vi "ZM-TST-pipeline.vi"() -> (0 "error out":errorcluster, 3 "Pass":bool)   [LabVIEW 2020, in "ZM-TST-tests.lvlib"]
doc: "T6, the data path without actors: simulated hardware into a file logger for 10 packages, after which TestPackage.jsonl holds 10 valid lines (pipeline_ok); with the placeholder hardware the first do fails and nothing is written (error_stops_ok). Pass = AND of both. Side effect: two temp folders under output."
uses:
  ZM-TST-tests.lvlib
  hardware/ZM-HW-SIM-simulated_hardware/ZM-HW-SIM-simulated_hardware/ZM-HW-SIM-simulated_hardware.lvclass
  hardware/ZM-HW-hardware/ZM-HW-hardware/ZM-HW-hardware.lvclass
  protocol/ZM-CP-FL-file_logger/ZM-CP-FL-file_logger/ZM-CP-FL-file_logger.lvclass
panel:
  out "error_stops_ok":bool
  out "pipeline_ok":bool
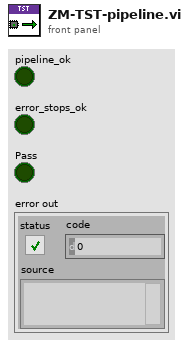
[diagram p1: front panel]
types:
  T1 = cluster{"timestamp":string, "type":string, "destination":string, "data":cluster{"temperature_c":dbl, "sample_index":i32, "duty_percent":u8, "sensor_ok":bool, "status":string}}
  T2 = cluster{"temperature_c":dbl, "sample_index":i32, "duty_percent":u8, "sensor_ok":bool, "status":string}
  T3 = cluster{"temperature_c":bool, "sample_index":bool, "duty_percent":bool, "sensor_ok":bool, "status":bool}
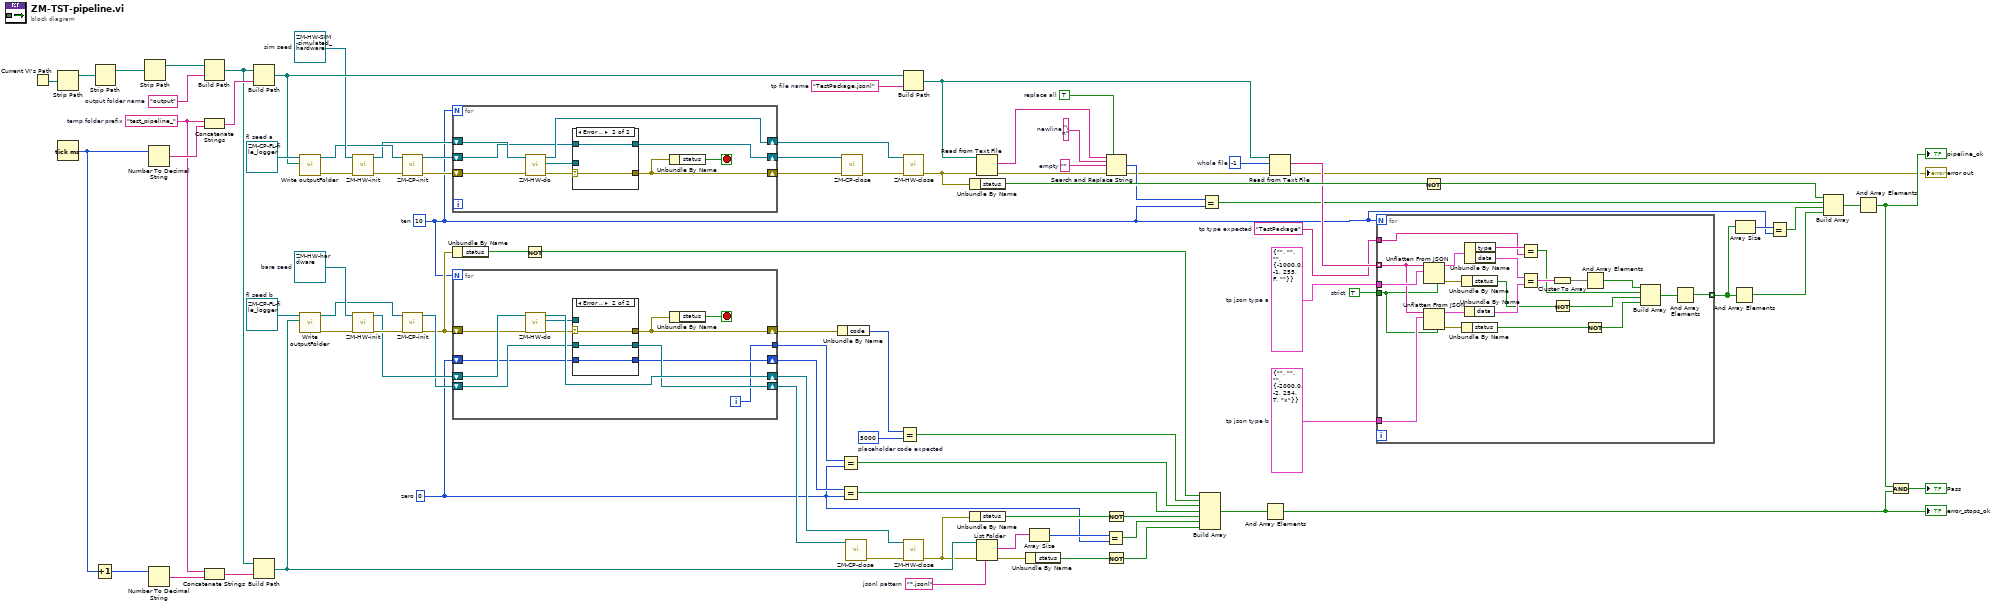
[diagram p0: block diagram]
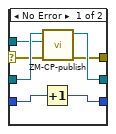
[diagram p2: hidden frame]
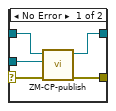
[diagram p3: hidden frame]
diagram:
  w15 = 0  # zero
  w18 = "*.jsonl"  # jsonl pattern
  w27 = 5000  # placeholder code expected
  w48 = TRUE  # strict
  w49 = T1 {"timestamp"="", "type"="", "destination"="", "data"={"temperature_c"=-2000.0, "sample_index"=-2, "duty_percent"=254, "sensor_ok"=TRUE, "status"="x"}}  # tp json type b
  w50 = T1 {"timestamp"="", "type"="", "destination"="", "data"={"temperature_c"=-1000.0, "sample_index"=-1, "duty_percent"=255, "sensor_ok"=FALSE, "status"=""}}  # tp json type a
  w30 = 10  # ten
  w53 = -1  # whole file
  w56 = TRUE  # replace all
  w58 = ""  # empty
  w59 = "\n"  # newline
  w47 = "TestPackage"  # tp type expected
  w76 = "TestPackage.jsonl"  # tp file name
  w86 = "test_pipeline_"  # temp folder prefix
  w80 = "output"  # output folder name
  w39 = refnum<class "ZM-CP-FL-file_logger.lvclass"> refnum  # fl seed b
  w75 = refnum<class "ZM-CP-FL-file_logger.lvclass"> refnum  # fl seed a
  w38 = refnum<class "ZM-HW-hardware.lvclass"> refnum  # bare seed
  w73 = refnum<class "ZM-HW-SIM-simulated_hardware.lvclass"> refnum  # sim seed
  n1 = Current VI's Path() -> (path=w84:path)
  n2 = Strip Path(path=w84) -> (stripped path=w83:path)  [unwired: 1 out]
  n3 = Tick Count (ms)() -> (millisecond timer value=w88:u32)
  n4 = Increment(x=w88) -> (x+1=w87:u32)
  n5 = Strip Path(path=w83) -> (stripped path=w82:path)  [unwired: 1 out]
  n6 = Strip Path(path=w82) -> (stripped path=w81:path)  [unwired: 1 out]
  n7 = Number To Decimal String(number=w88) -> (decimal integer string=w89:string)  [unwired: 1 in]
  n8 = Number To Decimal String(number=w87) -> (decimal integer string=w85:string)  [unwired: 1 in]
  n9 = Build Path(base path=w81, name or relative path=w80) -> (appended path=w78:path)
  n10 = Concatenate Strings(w86, w89) -> (w79:string)
  n11 = Concatenate Strings(w86, w85) -> (w77:string)
  n12 = Build Path(base path=w78, name or relative path=w79) -> (appended path=w74:path)
  n13 = Build Path(base path=w78, name or relative path=w77) -> (appended path=w20:path)
  n14 = call "Write outputFolder.vi"("outputFolder"=w74, "ZM-CP-FL-file_logger in"=w75) -> ("error out"=w72:errorcluster, "ZM-CP-FL-file_logger out"=w71:refnum<class "ZM-CP-FL-file_logger.lvclass">)  [unwired: 8 in]
  n15 = call "Write outputFolder.vi"("outputFolder"=w20, "ZM-CP-FL-file_logger in"=w39) -> ("error out"=w37:errorcluster, "ZM-CP-FL-file_logger out"=w36:refnum<class "ZM-CP-FL-file_logger.lvclass">)  [unwired: 8 in]
  n16 = call-dynamic "ZM-HW-init.vi"("error in (no error)"=w72, "ZM-HW-hardware in"=w73) -> ("error out"=w70:errorcluster, "ZM-HW-hardware out"=w69:refnum<class "ZM-HW-SIM-simulated_hardware.lvclass">)  [unwired: 8 in]
  n17 = call-dynamic "ZM-HW-init.vi"("error in (no error)"=w37, "ZM-HW-hardware in"=w38) -> ("error out"=w35:errorcluster, "ZM-HW-hardware out"=w33:refnum<class "ZM-HW-hardware.lvclass">)  [unwired: 8 in]
  n18 = call-dynamic "ZM-CP-init.vi"("error in (no error)"=w70, "ZM-CP-FL-file_logger in"=w71) -> ("error out"=w67:errorcluster, "ZM-CP-FL-file_logger out"=w68:refnum<class "ZM-CP-FL-file_logger.lvclass">)  [unwired: 8 in]
  n19 = call-dynamic "ZM-CP-init.vi"("error in (no error)"=w35, "ZM-CP-FL-file_logger in"=w36) -> ("error out"=w31:errorcluster, "ZM-CP-FL-file_logger out"=w32:refnum<class "ZM-CP-FL-file_logger.lvclass">)  [unwired: 8 in]
  n20 = for {
    N: w30 -> [_]
    shift-right: [w96] -> w64
    shift-left: w69 -> [w98]
    shift-right: [w93] -> w66
    shift-left: w68 -> [w95]
    shift-right: [w91] -> w65
    shift-left: w67 -> [w97]
    stop <- w90 stop-if-true
    n21 = call-dynamic "ZM-HW-do.vi"("error in (no error)"=w97, "ZM-HW-hardware in"=w98) -> ("error out"=w92:errorcluster, "package"=w94:refnum<class "ZM-PC-package.lvclass">, "ZM-HW-hardware out"=w96:refnum<class "ZM-HW-SIM-simulated_hardware.lvclass">)  [unwired: 7 in]
    n22 = case shown="Error .." w92 {
      selector: w92 -> [w99 w104]
      tunnel: w95 -> [w103 w105]
      tunnel: w94 -> [w102 _]
      tunnel: [w101 w105] -> w93
      tunnel: [w100 w104] -> w91
      frame No Error {
        n23 = call-dynamic "ZM-CP-publish.vi"("error in (no error)"=w99, "package"=w102, "ZM-CP-FL-file_logger in"=w103) -> ("error out"=w100:errorcluster, "ZM-CP-FL-file_logger out"=w101:refnum<class "ZM-CP-FL-file_logger.lvclass">)  [unwired: 7 in]
      }
      frame Error {
      }
    }
    n24 = Unbundle By Name(w91) -> ("status"=w90:bool)
  }
  n25 = Unbundle By Name(w31) -> ("status"=w34:bool)
  n26 = for {
    N: w30 -> [_]
    shift-right: [w115] -> w23
    shift-left: w33 -> [w117]
    shift-right: [w111] -> w24
    shift-left: w32 -> [w114]
    shift-right: [w108] -> w29
    shift-left: w31 -> [w116]
    shift-right: [w110] -> w25
    shift-left: w15 -> [w112]
    tunnel: [w106] -> w26
    i -> [w106]
    stop <- w107 stop-if-true
    n27 = call-dynamic "ZM-HW-do.vi"("error in (no error)"=w116, "ZM-HW-hardware in"=w117) -> ("error out"=w109:errorcluster, "package"=w113:refnum<class "ZM-PC-package.lvclass">, "ZM-HW-hardware out"=w115:refnum<class "ZM-HW-hardware.lvclass">)  [unwired: 7 in]
    n28 = case shown="Error .." w109 {
      selector: w109 -> [w118 w125]
      tunnel: w114 -> [w124 w127]
      tunnel: w113 -> [w123 _]
      tunnel: w112 -> [w122 w126]
      tunnel: [w121 w127] -> w111
      tunnel: [w120 w125] -> w108
      tunnel: [w119 w126] -> w110
      frame No Error {
        n29 = Increment(x=w122) -> (x+1=w119:i32)
        n30 = call-dynamic "ZM-CP-publish.vi"("error in (no error)"=w118, "package"=w123, "ZM-CP-FL-file_logger in"=w124) -> ("error out"=w120:errorcluster, "ZM-CP-FL-file_logger out"=w121:refnum<class "ZM-CP-FL-file_logger.lvclass">)  [unwired: 7 in]
      }
      frame Error {
      }
    }
    n31 = Unbundle By Name(w108) -> ("status"=w107:bool)
  }
  n32 = Not(x=w34) -> (.not. x?=w12:bool)
  n33 = Unbundle By Name(w29) -> ("code"=w28:i32)
  n34 = Equal?(x=w26, y=w15) -> (x = y?=w10:bool)
  n35 = Equal?(x=w25, y=w15) -> (x = y?=w9:bool)
  n36 = call-dynamic "ZM-CP-close.vi"("error in (no error)"=w65, "ZM-CP-communication_protocol in"=w66) -> ("error out"=w63:errorcluster)  [unwired: 8 in, 1 out]
  n37 = call-dynamic "ZM-CP-close.vi"("ZM-CP-communication_protocol in"=w24) -> ("error out"=w22:errorcluster)  [unwired: 9 in, 1 out]
  n38 = Equal?(x=w28, y=w27) -> (x = y?=w11:bool)
  n39 = Build Path(base path=w74, name or relative path=w76) -> (appended path=w54:path)
  n40 = call-dynamic "ZM-HW-close.vi"("error in (no error)"=w63, "ZM-HW-hardware in"=w64) -> ("error out"=w61:errorcluster)  [unwired: 8 in, 1 out]
  n41 = call-dynamic "ZM-HW-close.vi"("error in (no error)"=w22, "ZM-HW-hardware in"=w23) -> ("error out"=w19:errorcluster)  [unwired: 8 in, 1 out]
  n42 = Unbundle By Name(w61) -> ("status"=w62:bool)
  n43 = Unbundle By Name(w19) -> ("status"=w21:bool)
  n44 = Read from Text File(file (use dialog)=w54, error in=w61) -> (text=w60:string, error out=w57:errorcluster)  [unwired: 2 in, 2 out]
  n45 = List Folder(path=w20, pattern=w18, error in=w19) -> (filenames=w17:string[], error out=w14:errorcluster)  [unwired: 1 in, 2 out]
  n46 = Unbundle By Name(w14) -> ("status"=w13:bool)
  n47 = Array Size(array=w17) -> (size(s)=w16:i32)
  n48 = Equal?(x=w16, y=w15) -> (x = y?=w7:bool)
  n49 = Not(x=w21) -> (.not. x?=w8:bool)
  n50 = Not(x=w13) -> (.not. x?=w6:bool)
  n51 = Search and Replace String(replace all?=w56, input string=w60, search string=w59, replace string=w58, error in=w57) -> (number of replacements=w55:i32, error out=w52:errorcluster)  [unwired: 3 in, 2 out]
  n52 = Build Array(w12, w11, w10, w9, w8, w7, w6) -> (w5:bool[])
  n53 = Equal?(x=w55, y=w30) -> (x = y?=w43:bool)
  n54 = And Array Elements(Boolean array=w5) -> (logical AND=w3:bool)
  "error_stops_ok" <- w3
  n55 = Read from Text File(file (use dialog)=w54, count=w53, error in=w52) -> (text=w51:string[], error out=→"error out":errorcluster)  [unwired: 1 in, 2 out]
  n56 = for {
    N: w30 -> [_]
    tunnel: w51 -> [w148] mode=indexing
    tunnel: w50 -> [w149]
    tunnel: w49 -> [w147]
    tunnel: w48 -> [w146]
    tunnel: w47 -> [w138]
    tunnel: [w128] -> w45 mode=indexing
    n57 = Unflatten From JSON(JSON string=w148, type and defaults=w149, strict validation? (F)=w146) -> (value=w145:T1, error out=w137:errorcluster)  [unwired: 4 in]
    n58 = Unflatten From JSON(JSON string=w148, type and defaults=w147, strict validation? (F)=w146) -> (value=w144:T1, error out=w136:errorcluster)  [unwired: 4 in]
    n59 = Unbundle By Name(w137) -> ("status"=w135:bool)
    n60 = Unbundle By Name(w136) -> ("status"=w134:bool)
    n61 = Unbundle By Name(w144) -> ("data"=w142:T2)
    n62 = Unbundle By Name(w145) -> ("type"=w139:string, "data"=w143:T2)
    n63 = Equal?(x=w139, y=w138) -> (x = y?=w132:bool)
    n64 = Equal?(x=w143, y=w142) -> (x = y?=w141:T3)
    n65 = Cluster To Array(cluster=w141) -> (array=w140:bool[])
    n66 = Not(x=w135) -> (.not. x?=w131:bool)
    n67 = And Array Elements(Boolean array=w140) -> (logical AND=w133:bool)
    n68 = Not(x=w134) -> (.not. x?=w130:bool)
    n69 = Build Array(w133, w132, w131, w130) -> (w129:bool[])
    n70 = And Array Elements(Boolean array=w129) -> (logical AND=w128:bool)
  }
  n71 = Not(x=w62) -> (.not. x?=w44:bool)
  n72 = And Array Elements(Boolean array=w45) -> (logical AND=w41:bool)
  n73 = Array Size(array=w45) -> (size(s)=w46:i32)
  n74 = Equal?(x=w46, y=w30) -> (x = y?=w42:bool)
  n75 = Build Array(w44, w43, w42, w41) -> (w40:bool[])
  n76 = And Array Elements(Boolean array=w40) -> (logical AND=w4:bool)
  "pipeline_ok" <- w4
  n77 = And(x=w4, y=w3) -> (x .and. y?=→"Pass":bool)
